vi "convert Axis Info Array to Cluster.vi"(8 "error in (no error)":errorcluster, 10 "Axis Info Array":string[](array[string]), 11 "3D Controller in":refnum<class "3D Controller.lvclass">) -> (0 "error out":errorcluster, 2 "Axis Parameter List":T1, 3 "3D Controller out":refnum<class "3D Controller.lvclass">)   [LabVIEW 2023, in "FCC 3D Controller for BS.lvlib" / "3D Controller.lvclass"]
uses:
  3D Controller.lvclass
  3D Controller.lvclass/3D Controller.ctl
  Type Definition/TYPE Axis Parameter List.ctl
  FCC 3D Controller for BS.lvlib
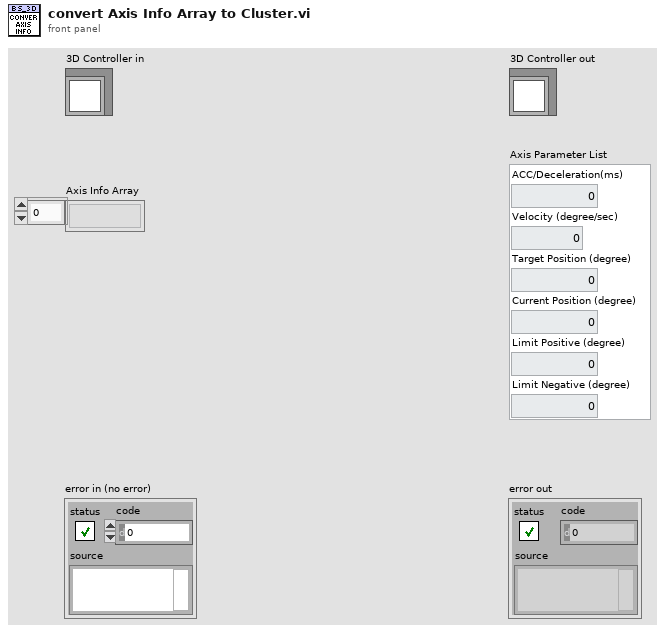
[diagram p1: front panel]
types:
  T1 = typedef "FCC 3D Controller for BS.lvlib/TYPE Axis Parameter List.ctl" = cluster{"ACC/Deceleration(ms)":dbl, "Velocity (degree/sec)":dbl, "Target Position (degree)":dbl, "Current Position (degree)":dbl, "Limit Positive (degree)":dbl, "Limit Negative (degree)":dbl}
  T2 = cluster{"[0]":dbl, "[1]":dbl, "[2]":dbl, "[3]":dbl, "[4]":dbl, "[5]":dbl}
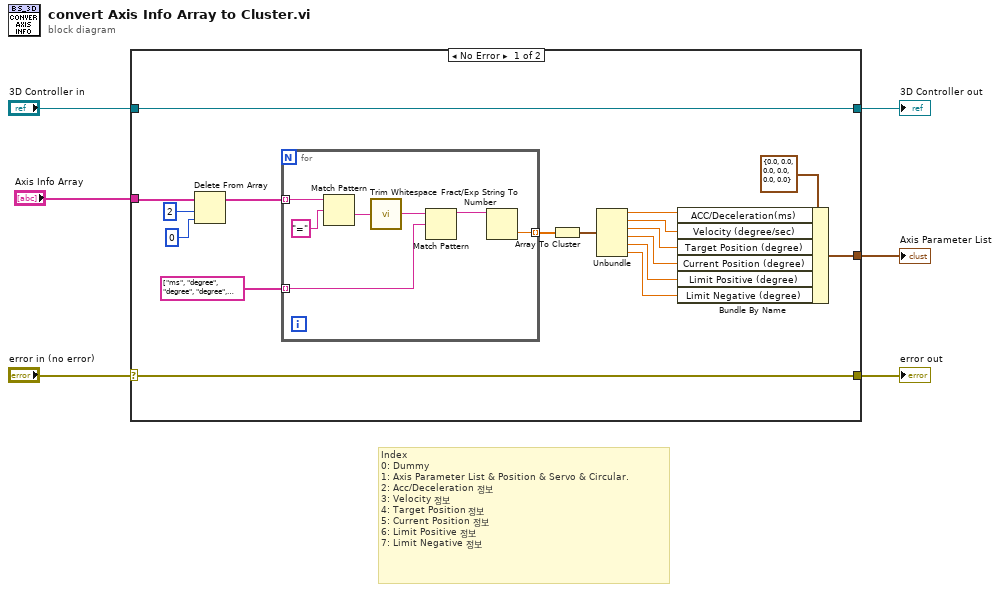
[diagram p0: block diagram]
diagram:
  # "Index\n0: Dummy\n1: Axis Parameter List & Position & Servo & Circular.\n2: Acc/Deceleration 정보\n3: Velocity 정보\n4: Target Position 정보\n5: Current Position 정보\n6: Limit Positive 정보\n7: Limit Negative 정보"
  n1 = case shown="No Error" "error in (no error)" {
    selector: "error in (no error)" -> [w22 w32]
    tunnel: [w22 w32] -> w5
    tunnel: [w23 w31] -> w3
    tunnel: "3D Controller in" -> [w23 w31]
    tunnel: "Axis Info Array" -> [w20 _]
    tunnel: [w7 _] -> w1
    frame No Error {
      n2 = Delete From Array(array=w20, length=2, index=0) -> (array with subset deleted=w17:string[])  [unwired: 1 out]
      n3 = for {
        tunnel: w17 -> [w30] mode=indexing
        tunnel: string[] ["ms", "degree", "degree", "degree", "degree", "degree"] ("regular expression") -> [w26] mode=indexing
        tunnel: [w24] -> w15 mode=indexing
        n4 = Match Pattern(string=w30, regular expression="=") -> (after substring=w28:string)  [unwired: 1 in, 3 out]
        n5 = call <vilib>:"Trim Whitespace.vi"("string"=w28) -> ("trimmed string"=w27:string)  [unwired: 1 in]
        n6 = Match Pattern(string=w27, regular expression=w26) -> (before substring=w25:string)  [unwired: 1 in, 3 out]
        n7 = Fract/Exp String To Number(string=w25) -> (number=w24:dbl)  [unwired: 3 in, 1 out]
      }
      n8 = Array To Cluster(array=w15) -> (cluster=w14:T2)
      n9 = Unbundle(w14) -> ("[0]"=w13:dbl, "[1]"=w12:dbl, "[2]"=w11:dbl, "[3]"=w10:dbl, "[4]"=w9:dbl, "[5]"=w8:dbl)
      n10 = Bundle By Name(cluster=T1 {"ACC/Deceleration(ms)"=0.0, "Velocity (degree/sec)"=0.0, "Target Position (degree)"=0.0, "Current Position (degree)"=0.0, "Limit Positive (degree)"=0.0, "Limit Negative (degree)"=0.0} ("Axis Parameter List 2"), "ACC/Deceleration(ms)"=w13, "Velocity (degree/sec)"=w12, "Target Position (degree)"=w11, "Current Position (degree)"=w10, "Limit Positive (degree)"=w9, "Limit Negative (degree)"=w8) -> (w7:T1)
    }
    frame Error {
    }
  }
  "error out" <- w5
  "3D Controller out" <- w3
  "Axis Parameter List" <- w1
